vi "Save Plot.vi"(6 "XY Plot":refnum<vi>, 8 "error in (no error)":errorcluster, 9 "TextBox position":cluster{"x":i16, "y":i16}={"x"=150, "y"=50}, 10 "Partnumber":string, 11 "XY Plotter":refnum<class "XY Plotter.lvclass">) -> (0 "error out":errorcluster, 3 "XY Plotter out":refnum<class "XY Plotter.lvclass">)   [LabVIEW 2025, in "XY Plotter.lvlib" / "XY Plotter.lvclass"]
uses:
  XY Plotter.lvclass
  XY Plotter.lvclass/XY Plotter.ctl
  XY Plotter configuration/XY Plotter configuration.lvclass/XY Plotter configuration.ctl
  XY Plotter configuration/Read XY Plotter.vi
  XY Plotter configuration/XY Plotter configuration.lvclass
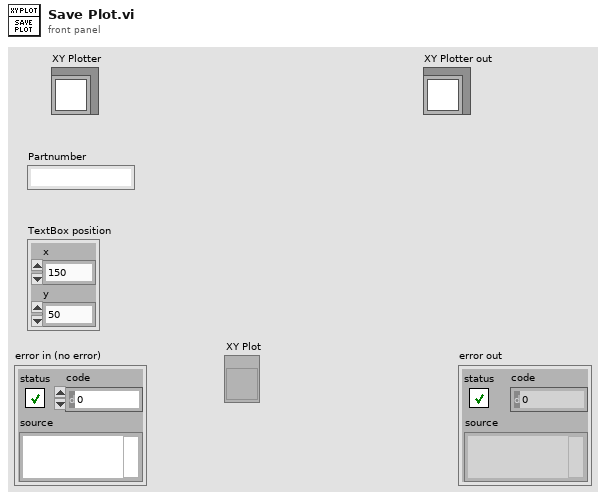
[diagram p1: front panel]
types:
  T1 = typedef "XY Plotter.lvlib/XY Plotter configuration.lvclass/XY Plotter.ctl" = cluster{"Data Rate":i32, "Y-Scales":cluster{"Label":string, "Max":dbl, "Min":dbl, "Unit":enum16{"---", "V", "mA", "sec", "dB", "deg", "in/s", "in", "lbf", "Hz", "psi", "gpm"}, "Visible":bool}[], "Note":string, "History Length":i32, "DataLog Path":path, "Plot type":bool, "X-Scales":cluster{"Label":string, "Max":dbl, "Min":dbl, "Unit":enum16{"---", "V", "mA", "sec", "dB", "deg", "in/s", "in", "lbf", "Hz", "psi", "gpm"}, "Visible":bool}[], "Plot List":cluster{"Plot Name":string, "X Scale Index":u32, "Y Scale Index":u32, "Visible":bool}[]}
  T2 = typedef "imagedata.ctl" = cluster{"image type":i32, "image depth":i32, "image":u8[], "mask":u8[], "colors":u32[], "Rectangle":cluster{"left":i16, "top":i16, "right":i16, "bottom":i16}}
  T3 = cluster{"Plot Name":string, "X Scale Index":u32, "Y Scale Index":u32, "Visible":bool}[]
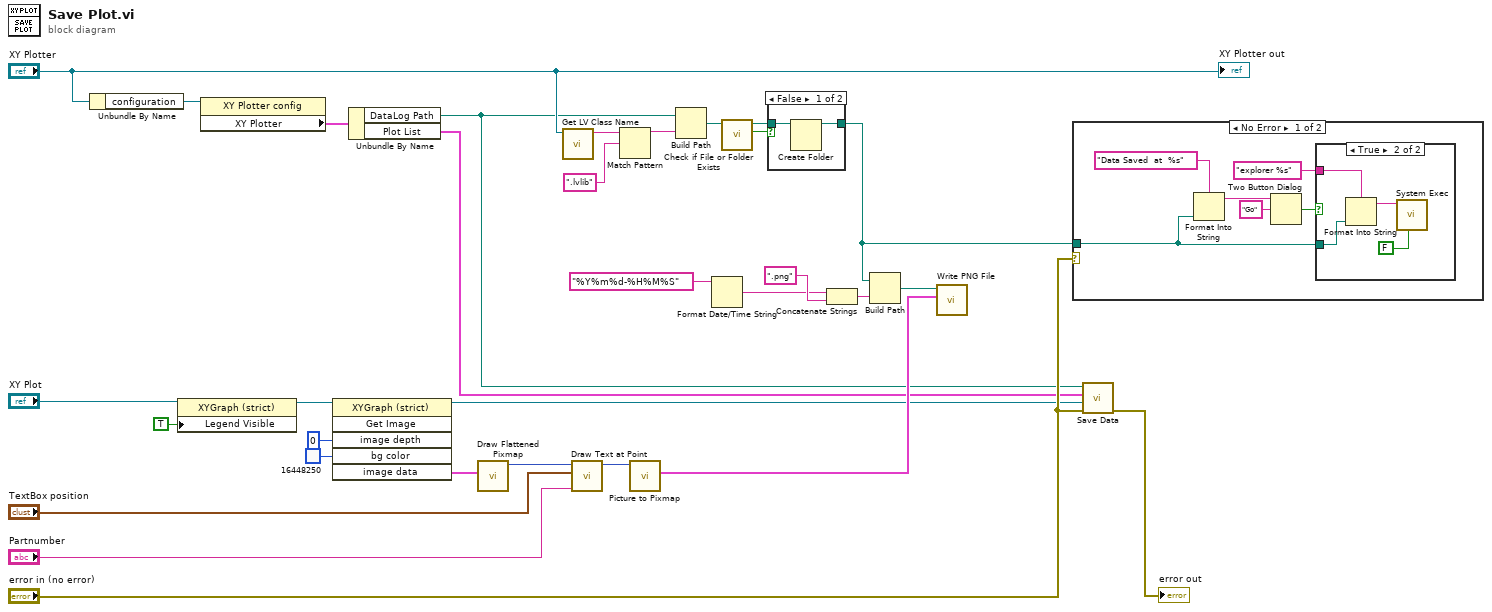
[diagram p0: block diagram]
diagram:
  n1 = Unbundle By Name("XY Plotter") -> ("configuration"=w4:refnum<class "XY Plotter configuration.lvclass">)
  n2 = property class="XYGraph (strict)"(reference="XY Plot", "Legend Visible"=TRUE ("Legend:Visible")) -> (reference out=w6:refnum<vi>)  [unwired: 1 in, 1 out]
  n3 = property class="XY Plotter config"(reference=w4) -> ("XY Plotter"=w17:T1)  [unwired: 1 in, 2 out]
  n4 = invoke class="XYGraph (strict)" method="Get Image"(reference=w6, "image depth"=0 ("Image Depth"), "bg color"=u32 16448250 ("Background Color")) -> (reference out=w5:refnum<vi>, "image data"=w27:T2)  [unwired: 3 in, 4 out]
  n5 = Unbundle By Name(w17) -> ("DataLog Path"=w3:path, "Plot List"=w2:T3)
  n6 = call <vilib>:"Draw Flattened Pixmap.vi"("image data"=w27) -> ("new picture"=w28:picture)  [unwired: 8 in]
  n7 = call <vilib>:"Get LV Class Name.vi"("object"="XY Plotter") -> ("class name"=w11:string)  [unwired: 9 in, 1 out]
  n8 = call <vilib>:"Draw Text at Point.vi"("text"="Partnumber", "origin"="TextBox position", "picture"=w28) -> ("new picture"=w29:picture)  [unwired: 7 in, 1 out]
  n9 = Match Pattern(string=w11, regular expression=".lvlib") -> (before substring=w10:string)  [unwired: 1 in, 3 out]
  n10 = call <vilib>:"Picture to Pixmap.vi"("picture"=w29) -> ("image data"=w26:T2)  [unwired: 9 in, 1 out]
  n11 = Build Path(base path=w3, name or relative path=w10) -> (appended path=w13:path)
  n12 = Format Date/Time String(time format string (%c)="%Y%m%d-%H%M%S") -> (date/time string=w24:string)  [unwired: 2 in]
  n13 = call <vilib>:"Check if File or Folder Exists.vi"("path"=w13) -> ("file or folder exists?"=w9:bool, "dup path"=w8:path)  [unwired: 8 in, 1 out]
  n14 = case shown="False" w9 {
    tunnel: w8 -> [w33 w34]
    tunnel: [w32 w34] -> w7
    frame False {
      n15 = Create Folder(path (use dialog)=w33) -> (created path=w32:path)  [unwired: 2 in, 2 out]
    }
    frame True {
    }
  }
  n16 = Concatenate Strings(w24, ".png" ("string")) -> (w23:string)
  n17 = Build Path(base path=w7, name or relative path=w23) -> (appended path=w20:path)
  n18 = call <vilib>:"Write PNG File.vi"("image data"=w26, "path to PNG file"=w20) -> ()  [unwired: 8 in, 2 out]
  n19 = case shown="No Error" "error in (no error)" {
    tunnel: w7 -> [w37 _]
    frame No Error {
      n20 = Format Into String(format string="Data Saved  at  %s", w37) -> (resulting string=w40:string)  [unwired: 2 in, 1 out]
      n21 = Two Button Dialog(message=w40, 2:"Go" ("T button name (\"OK\")")) -> (T button?=w38:bool)  [unwired: 1 in]
      n22 = case shown="True" w38 {
        tunnel: w37 -> [_ w43]
        tunnel: "explorer %s" ("command line") -> [_ w41]
        frame False {
        }
        frame True {
          n23 = Format Into String(format string=w41, w43) -> (resulting string=w42:string)  [unwired: 2 in, 1 out]
          n24 = call <vilib>:"System Exec.vi"("run minimized? (F)"=FALSE, "command line"=w42) -> ()  [unwired: 6 in, 4 out]
        }
      }
    }
    frame Error {
    }
  }
  n25 = call "Save Data.vi"("error in"="error in (no error)", "XY Plot"=w5, "Plot List"=w2, "DataLog Path"=w3) -> ("error out"=→"error out":errorcluster)  [unwired: 7 in]
  "XY Plotter out" <- "XY Plotter"
